vi "Cmd_Check.vi"(8 "error in":errorcluster, 11 "writer ref in":refnum<k21>) -> (0 "error out":errorcluster, 3 "disconnected?":bool)   [LabVIEW 2025]
uses:
  <resource>/objmgr/ni.dex.rc
  vi/thresholds.ctl
  vi/Command.ctl
  vi/RT_Cmd.ctl
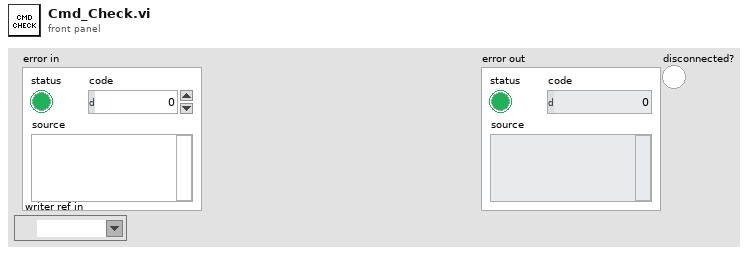
[diagram p1: front panel]
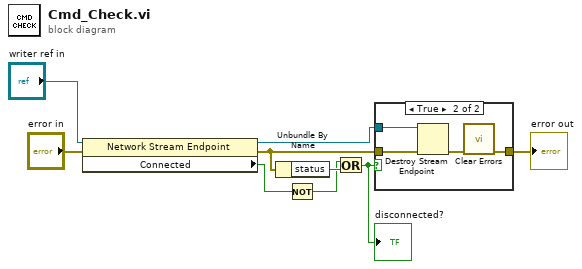
[diagram p0: block diagram]
diagram:
  n1 = property class="Network Stream Endpoint"(reference="writer ref in", error in="error in") -> (reference out=w6:refnum<k21>, error out=w5:errorcluster, "Connected"=w7:bool)
  n2 = Unbundle By Name(w5) -> ("status"=w4:bool)
  n3 = Not(x=w7) -> (.not. x?=w3:bool)
  n4 = Or(x=w3, y=w4) -> (x .or. y?=w1:bool)
  "disconnected?" <- w1
  n5 = case shown="True" w1 {
    tunnel: w6 -> [_ w14]
    tunnel: w5 -> [w10 w13]
    tunnel: [w10 w11] -> w2
    frame False {
    }
    frame True {
      n6 = Destroy Stream Endpoint(8:w13, 11:w14) -> (0:w12:errorcluster)
      n7 = call <vilib>:"Clear Errors.vi"("error in (no error)"=w12) -> ("error out"=w11:errorcluster)  [unwired: 5 in, 1 out]
    }
  }
  "error out" <- w2
